vi "cnm.vi"(8 "x":dbl) -> (0 "x+y":dbl)   [LabVIEW 2019]
panel:
  in  "s":bool
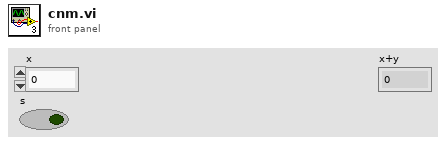
[diagram p1: front panel]
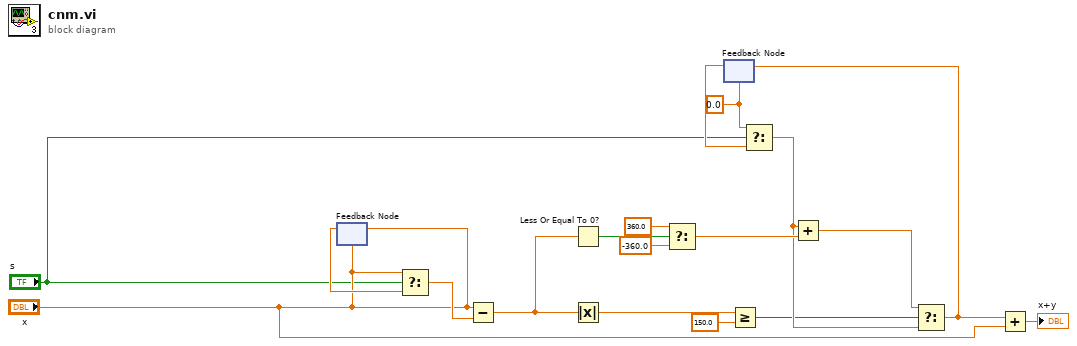
[diagram p0: block diagram]
diagram:
  w7 = 0.0 ("t")
  n1 = feedback #1("x") -> (w5:dbl)
  n2 = feedback-in #1("x") -> ()
  n3 = Select(t="x", s="s", f=w5) -> (s? t:f=w18:dbl)
  n4 = Subtract(x="x", y=w18) -> (x-y=w17:dbl)
  n5 = Less Or Equal To 0?(x=w17) -> (x <= 0?=w16:bool)
  n6 = Absolute Value(x=w17) -> (abs(x)=w9:dbl)
  n7 = Select(t=360.0, s=w16, f=-360.0) -> (s? t:f=w13:dbl)
  n8 = feedback #2(w7) -> (w6:dbl)
  n9 = Greater Or Equal?(x=w9, y=150.0) -> (x >= y?=w10:bool)
  n10 = Select(t=w7, s="s", f=w6) -> (s? t:f=w11:dbl)
  n11 = Add(x=w11, y=w13) -> (x+y=w12:dbl)
  n12 = Select(t=w12, s=w10, f=w11) -> (s? t:f=w4:dbl)
  n13 = feedback-in #2(w4) -> ()
  n14 = Add(x=w4, y="x") -> (x+y=→"x+y":dbl)
